vi "AO Echo Matches.vi"(8 "error in (no error)":errorcluster, 10 "AO Channel Echo":T1, 11 "Instrument.DAQ in":refnum<class "Instrument.DAQ.lvclass">) -> (0 "error out":errorcluster, 2 "keep?":bool, 3 "Instrument.DAQ out":refnum<class "Instrument.DAQ.lvclass">)   [LabVIEW 2019, in "Instrument.Lockin.lvlib" / "Instrument.DAQ.lvclass"]
uses:
  Instrument.DAQ.lvclass
  Generator/typedefs/AO.Channel--Cluster--Array.ctl
  Generator/typedefs/AO.Channel--Cluster.ctl
  Generator/typedefs/AO.Channel.Function--Enum.ctl
  Instrument.DAQ.lvclass/Instrument.DAQ.ctl
  Generator/Generator.lvclass
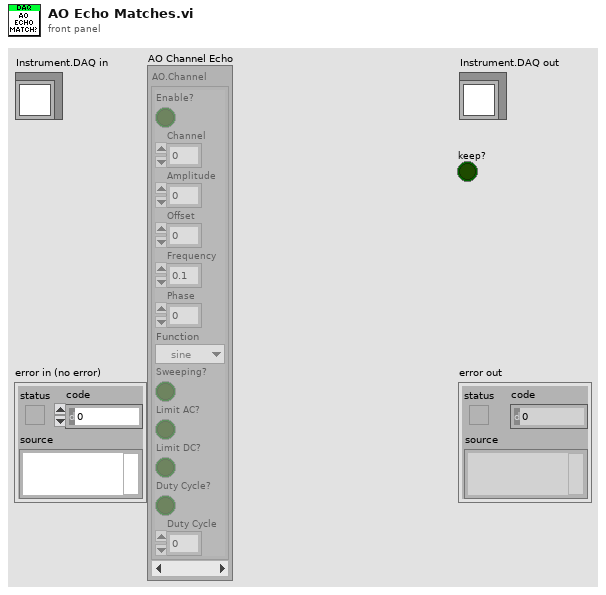
[diagram p1: front panel]
types:
  T1 = typedef "Generator.lvclass/AO.Channel--Cluster--Array.ctl" = T2[]
  T2 = typedef "Generator.lvclass/AO.Channel--Cluster.ctl" = cluster{"Enable?":bool, "Channel":i32, "Amplitude":dbl, "Offset":dbl, "Frequency":dbl, "Phase":dbl, "Function":T3, "Sweeping?":bool, "Limit AC?":bool, "Limit DC?":bool, "Duty Cycle?":bool, "Duty Cycle":dbl}
  T3 = typedef "Generator.lvclass/AO.Channel.Function--Enum.ctl" = enum16{"sine", "square", "triangle", "saw"}
  T4 = typedef "Instrument.Lockin.lvlib/Instrument.DAQ.lvclass/AO.Channel--Cluster--Array.ctl" = T5[]
  T5 = typedef "Instrument.Lockin.lvlib/Instrument.DAQ.lvclass/AO.Channel--Cluster.ctl" = cluster{"Enable?":bool, "Channel":i32, "Amplitude":dbl, "Offset":dbl, "Frequency":dbl, "Phase":dbl, "Function":T6, "Sweeping?":bool, "Limit AC":bool, "Limit DC?":bool, "Duty Cycle":bool}
  T6 = typedef "Instrument.Lockin.lvlib/Instrument.DAQ.lvclass/AO.Channel.Function--Enum.ctl" = enum16{"sine", "square", "triangle", "saw"}
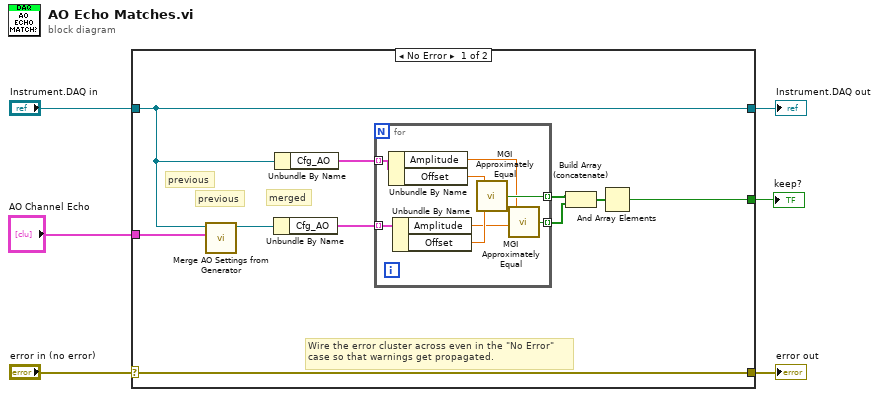
[diagram p0: block diagram]
diagram:
  n1 = case shown="No Error" "error in (no error)" {
    selector: "error in (no error)" -> [w16 w26]
    tunnel: [w16 w26] -> w5
    tunnel: [w13 w25] -> w3
    tunnel: "Instrument.DAQ in" -> [w13 w25]
    tunnel: "AO Channel Echo" -> [w15 _]
    tunnel: [w7 _] -> w1
    frame No Error {
      # "merged"
      # "previous"
      # "previous"
      # "Wire the error cluster across even in the \"No Error\"\ncase so that warnings get propagated."
      n2 = call "Merge AO Settings from Generator.vi"("configuration.AO Channels"=w15, "Instrument.DAQ in"=w13) -> ("Instrument.DAQ out"=w14:refnum<class "Instrument.DAQ.lvclass">)  [unwired: 8 in, 1 out]
      n3 = Unbundle By Name(w14) -> ("Cfg_AO"=w12:T4)
      n4 = Unbundle By Name(w13) -> ("Cfg_AO"=w11:T4)
      n5 = for {
        tunnel: w12 -> [w23] mode=indexing
        tunnel: w11 -> [w24] mode=indexing
        tunnel: [w20] -> w9 mode=indexing
        tunnel: [w19] -> w10 mode=indexing
        n6 = Unbundle By Name(w24) -> ("Amplitude"=w18:dbl, "Offset"=w17:dbl)
        n7 = Unbundle By Name(w23) -> ("Amplitude"=w21:dbl, "Offset"=w22:dbl)
        n8 = call <userlib>:"MGI Approximately Equal.vi"("Numeric 2"=w22, "Numeric 1"=w17) -> ("approx = ?"=w20:bool)
        n9 = call <userlib>:"MGI Approximately Equal.vi"("Numeric 2"=w21, "Numeric 1"=w18) -> ("approx = ?"=w19:bool)
      }
      n10 = Build Array (concatenate)(w9, w10) -> (w8:bool[])
      n11 = And Array Elements(Boolean array=w8) -> (logical AND=w7:bool)
    }
    frame Error {
    }
  }
  "error out" <- w5
  "Instrument.DAQ out" <- w3
  "keep?" <- w1
